vi "Register HTTP.vi"(8 "error in (no error)":errorcluster, 11 "Volatus Core in":refnum<class "Volatus Core.lvclass">) -> (0 "error out":errorcluster, 3 "Volatus Core out":refnum<class "Volatus Core.lvclass">)   [LabVIEW 2020, in "Volatus.lvlib" / "Volatus Core.lvclass"]
uses:
  Volatus Core.lvclass
  C:/dev/lv20CE/relink/lv-volatus/Volatus/Module/Module.lvclass
  Module/Module.lvclass/Module.ctl
  Config Type.ctl
  Volatus Core.lvclass/Volatus Core.ctl
  VolatusApiHttpService/VolatusApiHttpService.lvclass
  C:/dev/lv20CE/relink/lv-http-server/HTTP Server/Service/Service.lvclass
  DebugHTTPController/DebugHTTPController.lvclass
  C:/dev/lv20CE/relink/lv-http-server/HTTP Server/Handler/Handler.lvclass
  VolatusVariableResolver/VolatusVariableResolver.lvclass
  C:/dev/lv20CE/relink/lv-http-server/HTTP Server/TemplateVariableResolver/TemplateValueResolver.lvclass
  lv-http-server/HTTP Server/BasicTemplater/BasicTemplater.lvclass
  C:/dev/lv20CE/relink/lv-http-server/HTTP Server/TemplateService/TemplateService.lvclass
  lv-http-server/HTTP Server/Server/Add Connection Handler.vi
  lv-http-server/HTTP Server/Server/Add Request Handler.vi
  lv-http-server/HTTP Server/Server/Add Route Handler.vi
  lv-http-server/HTTP Server/Server/Add Controller Handler.vi
  lv-http-server/HTTP Server/Server/Add Controller.vi
  lv-http-server/HTTP Server/Server/Add Response Handler.vi
  lv-http-server/HTTP Server/Server/Add Complete Handler.vi
  lv-http-server/HTTP Server/Server/Add Exception Handler.vi
  lv-http-server/HTTP Server/Connection Handler/Connection Handler.lvclass
  lv-http-server/HTTP Server/Request Handler/Request Handler.lvclass
  lv-http-server/HTTP Server/Route Handler/Route Handler.lvclass
  lv-http-server/HTTP Server/Controller Handler/Controller Handler.lvclass
  lv-http-server/HTTP Server/Controller/Controller.lvclass
  lv-http-server/HTTP Server/Response Handler/Response Handler.lvclass
  lv-http-server/HTTP Server/Complete Handler/Complete Handler.lvclass
  lv-http-server/HTTP Server/Exception Handler/Exception Handler.lvclass
  lv-http-server/HTTP Server/Handler/Handler.lvclass
  Module/Module.lvclass
  VolatusAPI/VolatusAPI.lvclass
  HTTP Manager/HTTP Manager.lvclass
  lv-http-server/HTTP Server/Server/Server.lvclass
  Nav Route/Nav Route.lvclass
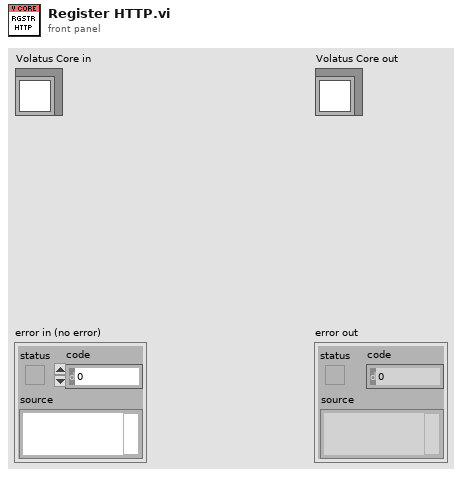
[diagram p1: front panel]
types:
  T1 = typedef "Volatus.lvlib/Volatus Core.lvclass/Config Type.ctl" = enum16{"App INI", "Memory", "Unconfigured"}
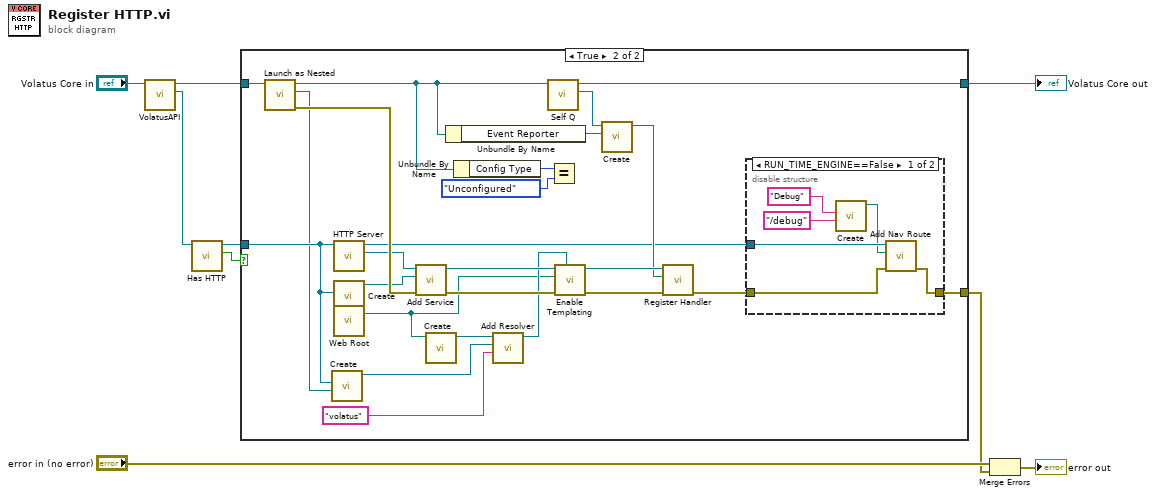
[diagram p0: block diagram]
diagram:
  n1 = call "VolatusAPI.vi"("Module in"="Volatus Core in") -> ("VolatusAPI"=w8:refnum<class "VolatusAPI.lvclass">, "Module out"=w5:refnum<class "Volatus Core.lvclass">)  [unwired: 9 in]
  n2 = call "Has HTTP.vi"("VolatusAPI in"=w8) -> ("Has HTTP"=w6:bool, "VolatusAPI out"=w4:refnum<class "VolatusAPI.lvclass">)  [unwired: 9 in]
  n3 = case shown="True" w6 {
    tunnel: w5 -> [w10 w31]
    tunnel: w4 -> [_ w21]
    tunnel: [w10 w29] -> w3
    tunnel: [_ w13] -> w1
    frame False {
    }
    frame True {
      n4 = call "Launch as Nested.vi"("Parent in"=w31) -> ("error out"=w34:errorcluster, "MessageQ"=w16:refnum<class "MessageQ.lvclass">, "Parent"=w27:refnum<class "Volatus Core.lvclass">)  [unwired: 8 in]
      n5 = call "Create.vi"("HTTP Manager"=w16, "VolatusAPI"=w21) -> ("VolatusVariableResolver out"=w19:refnum<class "VolatusVariableResolver.lvclass">)  [unwired: 8 in, 1 out]
      n6 = call "HTTP Server.vi"("VolatusAPI in"=w21) -> ("HTTP"=w26:refnum<class "Server.lvclass">, "VolatusAPI out"=w15:refnum<class "VolatusAPI.lvclass">)  [unwired: 9 in]
      n7 = call "Create.vi"("VolatusAPI"=w21) -> ("VolatusApiHttpService out"=w25:refnum<class "VolatusApiHttpService.lvclass">)  [unwired: 10 in]
      n8 = call "Web Root.vi"() -> ("WWW Root"=w12:path)  [unwired: 7 in]
      n9 = call "Add Service.vi"("error in (no error)"=w34, "Service"=w25, "Server in"=w26) -> ("error out"=w35:errorcluster, "Server out"=w24:refnum<class "Server.lvclass">)  [unwired: 7 in]
      n10 = call "Create.vi"("Templates Root"=w12) -> ("BasicTemplater out"=w20:refnum<class "BasicTemplater.lvclass">)  [unwired: 9 in, 1 out]
      n11 = Unbundle By Name(w27) -> ("Event Reporter"=w30:refnum<class "MessageQ.lvclass">)
      n12 = Unbundle By Name(w27) -> ("Config Type"=w33:T1)
      n13 = call "Add Resolver.vi"("Namespace"="volatus" ("Default Namespace"), "Resolver"=w19, "BasicTemplater in"=w20) -> ("BasicTemplater out"=w18:refnum<class "BasicTemplater.lvclass">)  [unwired: 7 in, 1 out]
      n14 = call "Self Q.vi"("Module in"=w27) -> ("Self Q"=w28:refnum<class "MessageQ.lvclass">, "Module out"=w29:refnum<class "Volatus Core.lvclass">)  [unwired: 9 in]
      n15 = Equal?(x=w33, y=Config_Type."Unconfigured") -> ()  [unwired: 1 out]
      n16 = call "Enable Templating.vi"("TemplateService (Basic)"=w18, "error in (no error)"=w35, "Root Folder"=w12, "Server in"=w24) -> ("error out"=w17:errorcluster, "Server out"=w23:refnum<class "Server.lvclass">)  [unwired: 6 in]
      n17 = call "Create.vi"("Event Module Q"=w30, "Core Module Q"=w28) -> ("DebugHTTPController out"=w22:refnum<class "DebugHTTPController.lvclass">)  [unwired: 8 in, 1 out]
      n18 = call "Register Handler.vi"("error in (no error)"=w17, "Handler"=w22, "Server in"=w23) -> ("error out"=w14:errorcluster)  [unwired: 7 in, 1 out]
      n19 = disable-structure shown="RUN_TIME_ENGINE==False" {
        disable-tunnel: w15 -> [w41 _]
        disable-tunnel: w14 -> [w40 w42]
        disable-tunnel: [w39 w42] -> w13
        frame condition #0 (active) {
          n20 = call "Create.vi"("Path"="/debug", "Label"="Debug") -> ("Nav Route out"=w36:refnum<class "Nav Route.lvclass">)  [unwired: 8 in, 1 out]
          n21 = call "Add Nav Route.vi"("error in (no error)"=w40, "Nav Route"=w36, "VolatusAPI in"=w41) -> ("error out"=w39:errorcluster)  [unwired: 7 in, 1 out]
        }
        frame condition #1 {
        }
      }
    }
  }
  "Volatus Core out" <- w3
  n22 = Merge Errors("error in (no error)", w1) -> (→"error out":errorcluster)
